vi "Parse GET Object Result.vi"(11 "Response header":string) -> (2 "User-Defined Metadata":T1[](array[typedef]), 3 "Get Object Result":T2)   [LabVIEW 2015, in "NI_AWS_S3.lvlib" / "Object.lvlib"]
uses:
  Object.lvlib
  GET Object Result Parameters.ctl
  Core/HTTP Request/Name Value Pair.ctl
  NI_AWS_S3.lvlib
  Core/NI_AWS_Core.lvlib
  Core/HTTP Request/HTTP Request.lvclass
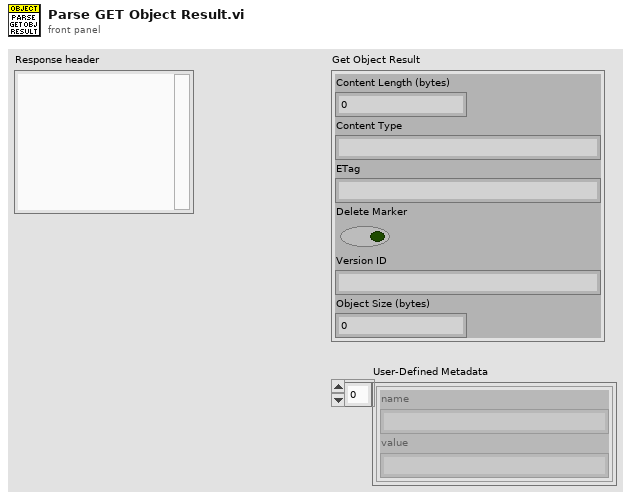
[diagram p1: front panel]
types:
  T1 = typedef "NI_AWS_Core.lvlib/HTTP Request.lvclass/Name Value Pair.ctl" = cluster{"name":string, "value":string}
  T2 = typedef "NI_AWS_S3.lvlib/GET Object Result Parameters.ctl" = cluster{"Content Length (bytes)":u64, "Content Type":string, "ETag":string, "Delete Marker":bool, "Version ID":string, "Object Size (bytes)":u64}
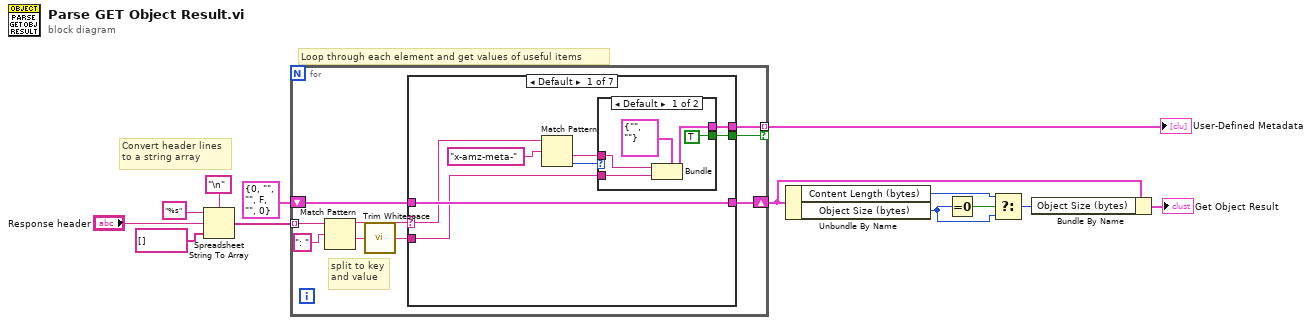
[diagram p0: block diagram]
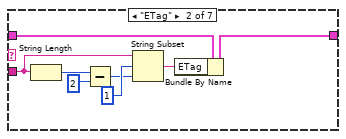
[diagram p3: hidden frame]
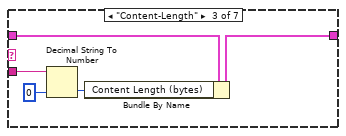
[diagram p4: hidden frame]
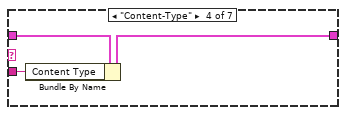
[diagram p5: hidden frame]
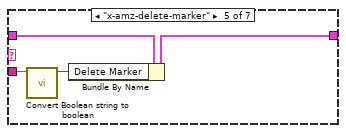
[diagram p6: hidden frame]
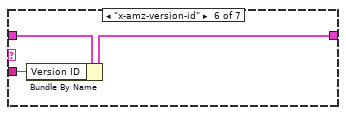
[diagram p7: hidden frame]
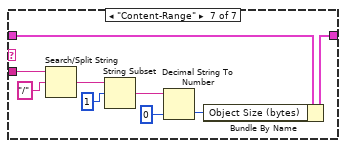
[diagram p8: hidden frame]
diagram:
  # "Loop through each element and get values of useful items"
  # "Convert header lines\nto a string array"
  n1 = Spreadsheet String To Array(delimiter (Tab)="\n", format string="%s", spreadsheet string="Response header", array type (2D Dbl)=string[] []) -> (array=w10:string[])
  n2 = for {
    tunnel: w10 -> [w22] mode=indexing
    shift-right: [w18] -> w4
    shift-left: T2 {"Content Length (bytes)"=0, "Content Type"="", "ETag"="", "Delete Marker"=FALSE, "Version ID"="", "Object Size (bytes)"=0} ("GetObjectResult") -> [w19]
    tunnel: [w15] -> w1 mode=indexing if=w14
    # "split to key\nand value"
    n3 = Match Pattern(string=w22, regular expression=": ") -> (before substring=w20:string, after substring=w17:string)  [unwired: 1 in, 2 out]
    n4 = call <vilib>:"Trim Whitespace.vi"("string"=w17) -> ("trimmed string"=w16:string)  [unwired: 1 in]
    n5 = case shown="Default" w20 {
      selector: w20 -> [w27 _ _ _ _ _ _]
      tunnel: w16 -> [w26 w42 w48 w50 w53 w56 w63]
      tunnel: w19 -> [w30 w38 w46 w51 w55 w58 w62]
      tunnel: [w30 w36 w44 w49 w54 w57 w61] -> w18
      tunnel: [w24 _ _ _ _ _ _] -> w15
      tunnel: [w23 _ _ _ _ _ _] -> w14
      frame Default {
        n6 = Match Pattern(string=w27, regular expression="x-amz-meta-") -> (after substring=w28:string, offset past match=w29:i32)  [unwired: 1 in, 2 out]
        n7 = case shown="Default" w29 {
          tunnel: w28 -> [w35 _]
          tunnel: w26 -> [w34 _]
          tunnel: [w32 _] -> w24
          tunnel: [TRUE _] -> w23
          frame Default {
            n8 = Bundle(cluster=T1 {"name"="", "value"=""} ("Name Value Pair"), "name"=w35, "value"=w34) -> (w32:T1)
          }
          frame -1 {
          }
        }
      }
      frame "ETag" {
        n9 = String Length(string=w42) -> (length=w41:i32)
        n10 = Subtract(x=w41, y=2) -> (x-y=w40:i32)
        n11 = String Subset(string=w42, offset (0)=1, length (rest)=w40) -> (substring=w37:string)
        n12 = Bundle By Name(cluster=w38, "ETag"=w37) -> (w36:T2)
      }
      frame "Content-Length" {
        n13 = Decimal String To Number(string=w48, default (0L)=u64 0 ("default (0 I32)")) -> (number=w45:u64)  [unwired: 1 in, 1 out]
        n14 = Bundle By Name(cluster=w46, "Content Length (bytes)"=w45) -> (w44:T2)
      }
      frame "Content-Type" {
        n15 = Bundle By Name(cluster=w51, "Content Type"=w50) -> (w49:T2)
      }
      frame "x-amz-delete-marker" {
        n16 = call "Convert Boolean string to boolean.vi"("Boolean String"=w53) -> ("Boolean"=w52:bool)  [unwired: 10 in]
        n17 = Bundle By Name(cluster=w55, "Delete Marker"=w52) -> (w54:T2)
      }
      frame "x-amz-version-id" {
        n18 = Bundle By Name(cluster=w58, "Version ID"=w56) -> (w57:T2)
      }
      frame "Content-Range" {
        n19 = Search/Split String(string=w63, search string/char (-)="/") -> (match + rest of string=w66:string)  [unwired: 1 in, 2 out]
        n20 = String Subset(string=w66, offset (0)=1) -> (substring=w64:string)  [unwired: 1 in]
        n21 = Decimal String To Number(string=w64, default (0L)=u64 0) -> (number=w60:u64)  [unwired: 1 in, 1 out]
        n22 = Bundle By Name(cluster=w62, "Object Size (bytes)"=w60) -> (w61:T2)
      }
    }
  }
  "User-Defined Metadata" <- w1
  n23 = Unbundle By Name(w4) -> ("Content Length (bytes)"=w6:u64, "Object Size (bytes)"=w5:u64)
  n24 = Equal To 0?(x=w5) -> (x = 0?=w7:bool)
  n25 = Select(t=w6, s=w7, f=w5) -> (s? t:f=w3:u64)
  n26 = Bundle By Name(cluster=w4, "Object Size (bytes)"=w3) -> (→"Get Object Result":T2)
